vi "SA set Marker Auto MAX.vi"(8 "error in (no error)":errorcluster caption="에러 입력(에러 없음)", 10 "Marker Index":i32, 11 "Instrument Manager 입력":refnum<class "Instrument Manager.lvclass">) -> (0 "error out":errorcluster caption="에러 출력", 3 "Instrument Manager 출력":refnum<class "Instrument Manager.lvclass">)   [LabVIEW 2023, in "Instrument Manager.lvclass"]
uses:
  Instrument Manager.lvclass
  Instrument Manager.lvclass/Instrument Manager.ctl
  Module/Spectrum Analyzer/Class/FSV-40N/FSV-40N.lvclass
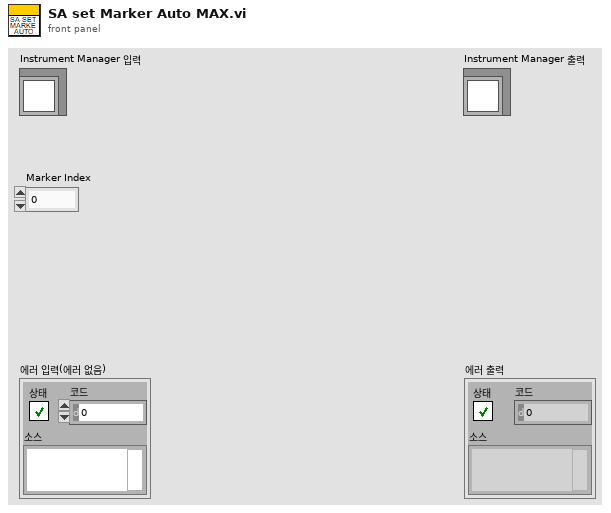
[diagram p1: front panel]
types:
  T1 = cluster{"Anritsu Call Box":refnum<class "Anritsu Call Box.lvclass">, "Spectrum Analyzer":refnum<class "Interface_Spectrum.lvclass">, "RF Switch Box":refnum<class "RF Filter Box.lvclass">, "Turn Table":refnum<class "Interface - Turn Table.lvclass">, "Mast":refnum<class "Interface - Mast.lvclass">, "3D Controller":refnum<class "Interface_3D Controller.lvclass">}
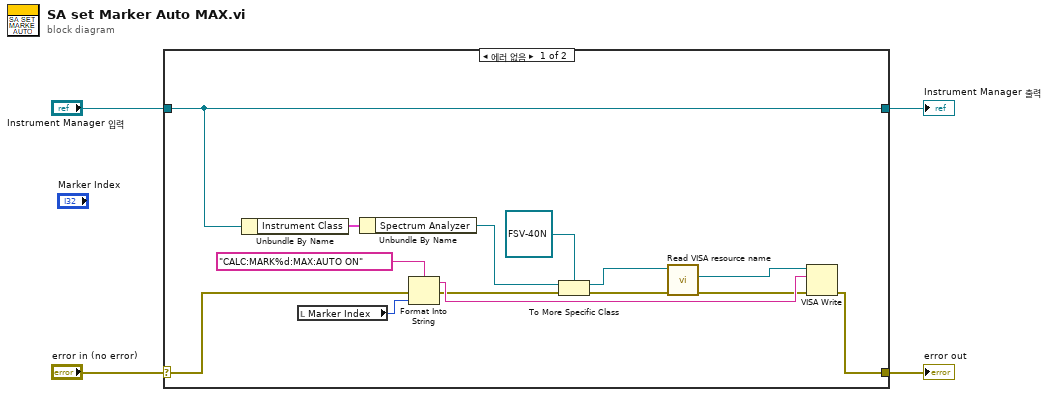
[diagram p0: block diagram]
diagram:
  n1 = case shown="에러 없음" "error in (no error)" {
    selector: "error in (no error)" -> [w6 w20]
    tunnel: [w5 w20] -> w3
    tunnel: [w7 w19] -> w1
    tunnel: "Instrument Manager 입력" -> [w7 w19]
    frame No Error {
      n2 = Unbundle By Name(w7) -> ("Instrument Class"=w10:T1)
      n3 = local read "Marker Index"() -> (w17:i32)
      n4 = Unbundle By Name(w10) -> ("Spectrum Analyzer"=w16:refnum<class "Interface_Spectrum.lvclass">)
      n5 = Format Into String(format string="CALC:MARK%d:MAX:AUTO ON" ("initial string"), error in=w6, w17) -> (resulting string=w18:string, error out=w11:errorcluster)  [unwired: 1 in]
      n6 = To More Specific Class(target class=refnum<class "FSV-40N.lvclass"> refnum ("Spectrum Analyzer.lvlib:FSV-40N.lvclass"), reference=w16, error in=w11) -> (specific class reference=w13:refnum<class "FSV-40N.lvclass">, error out=w12:errorcluster)
      n7 = call "Read VISA resource name.vi"("error in (no error)"=w12, "FSV-40N in"=w13) -> ("error out"=w14:errorcluster, "VISA resource name"=w15:refnum<visa-resource-name>)  [unwired: 7 in, 1 out]
      n8 = VISA Write(VISA resource name=w15, write buffer=w18, error in (no error)=w14) -> (error out=w5:errorcluster)  [unwired: 2 out]
    }
    frame Error {
    }
  }
  "error out" <- w3
  "Instrument Manager 출력" <- w1
